vi "SensorDetect.vi"(0 "Threshold":sgl=20.0, 2 "NXT/EV3 IN":T2, 3 "Port (Port 1)":T1 items=["Port 1", "Port 2", "Port 3", "Port 4"]) -> (1 "Out":bool, 4 "NXT/EV3 OUT":T2)   [LabVIEW 2016, in "13.03 Robot.lvrbt"]
uses:
  13.03 Robot.lvrbt
  <vilib>/NXT/Subs/LVHSConnector.ctl
  <vilib>/NXT/LegoClasses/BrickReference/BrickReference.lvclass
  <vilib>/NXT/Block Support/NXT_InputPort.ctl
  <vilib>/NXT/Dual Mode Library/Sensors/EV3_Color_Reflect.vi
  <vilib>/NXT/Dual Mode Library/Display/drawNumber.vi
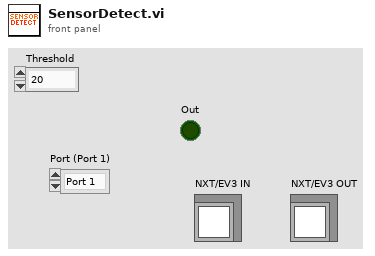
[diagram p1: front panel]
types:
  T1 = typedef "NXT_InputPort.ctl" = u32
  T2 = typedef "LVHSConnector.ctl" = refnum<class "BrickReference.lvclass">
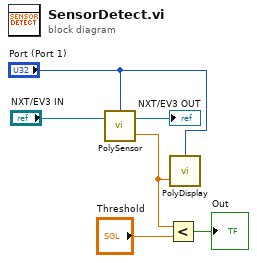
[diagram p0: block diagram]
diagram:
  n1 = call-poly <vilib>:"PolySensor.vi"("NXT/EV3"="NXT/EV3 IN", "Port (Port 1)"="Port (Port 1)") -> ("Scaled Value"=w1:sgl, "NXT/EV3"=→"NXT/EV3 OUT":T2)  [unwired: 1 in]
  n2 = Less?(x=w1, y="Threshold") -> (x < y?=→"Out":bool)
  n3 = call-poly <vilib>:"PolyDisplay.vi"("number"=w1, "Line"="Port (Port 1)") -> ()  [unwired: 2 in, 1 out]
